vi "Create Error (ID).vi"(4 "timestamp? (True)":bool=TRUE, 5 "is warning? (False)":bool, 6 "error override? (False)":bool, 7 "arg. call chain? (True)":bool=TRUE, 8 "error in (no error)":errorcluster, 9 "error arguments (\"\")":string, 10 "error description (\"\")":string, 11 "error id":string) -> (0 "error out":errorcluster)   [LabVIEW 2019, in "Error Generation.lvlib"]
doc: "Creates an error with an error ID instead of an error code. (Internally code = 637237 is used)\nThis function is similar to original NI \"Error Cluster From Error Code.vi\". Additional functions:\n<b>timestamp?</b>\nadd a current date & time string to the error description.\n<b>error override?</b>\nOverride the error on the input with the error code, despriction & arguments. \n<b>error arguments</b>\nInsert an argument name and data in this format: argument=argument data\nMultiple Arguments can be inserted EOL separated.\nUse arguments, to specify the error more detailled.\n- - -\nCopyright (c) 2023, Merecs Engineering GmbH"
uses:
  Error Generation.lvlib
  <vilib>/Utility/error.llb/Clear Errors.vi
  support/Convert Argument Representation.vi
  support/Search and Replace String With Arguments.vi
  Add Error Description.vi
  Get Argument.vi
  support/Is Error Code.vi
  support/Error Cluster From Error Code (Merecs).vi
  String to Match Pattern Case Insensitive.vi
  <vilib>/Utility/error.llb/Trim Whitespace.vi
  <vilib>/Utility/error.llb/Check Special Tags.vi
panel:
  # "Connector Pane"
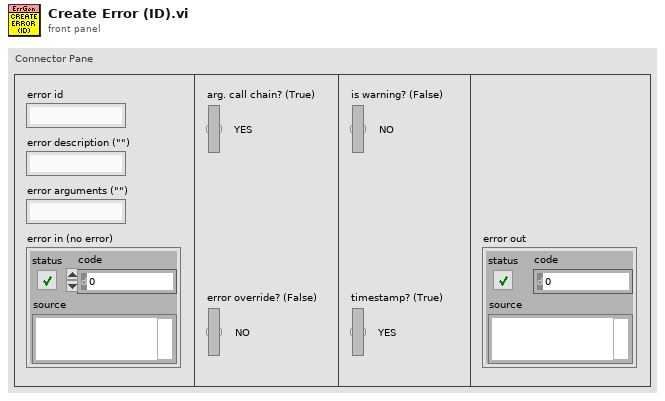
[diagram p1: front panel]
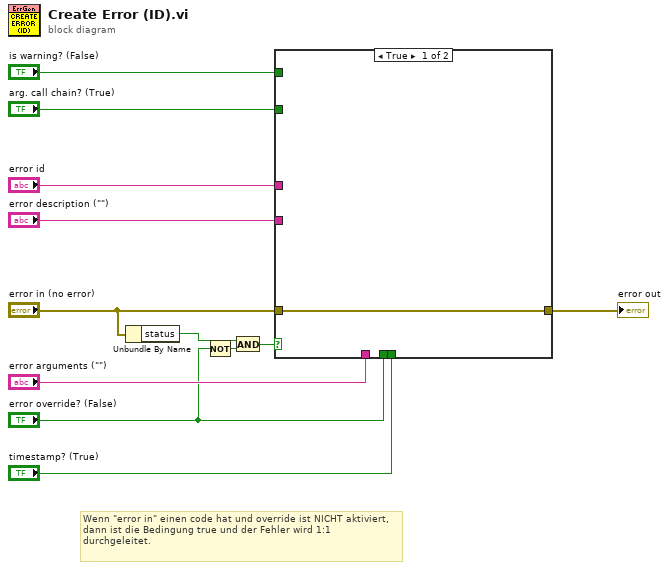
[diagram p0: block diagram]
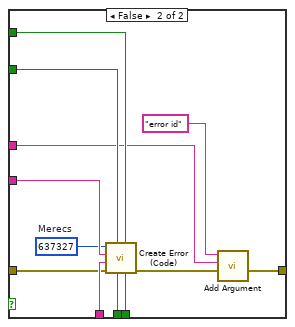
[diagram p2: hidden frame]
diagram:
  # "Wenn \"error in\" einen code hat und override ist NICHT aktiviert, dann ist die Bedingung true und der Fehler wird 1:1 durchgeleitet."
  n1 = Unbundle By Name("error in (no error)") -> ("status"=w4:bool)
  n2 = Not(x="error override? (False)") -> (.not. x?=w2:bool)
  n3 = And(x=w4, y=w2) -> (x .and. y?=w1:bool)
  n4 = case shown="True" w1 {
    tunnel: "error arguments (\"\")" -> [_ w24]
    tunnel: "error description (\"\")" -> [_ w23]
    tunnel: "error override? (False)" -> [_ w22]
    tunnel: "timestamp? (True)" -> [_ w21]
    tunnel: "arg. call chain? (True)" -> [_ w19]
    tunnel: "is warning? (False)" -> [_ w18]
    tunnel: "error in (no error)" -> [w13 w17]
    tunnel: [w13 w16] -> w7
    tunnel: "error id" -> [_ w15]
    frame True {
    }
    frame False {
      w20 = 637327  # Merecs
      n5 = call "Create Error (Code).vi"("timestamp? (True)"=w21, "is warning? (False)"=w18, "error override? (True)"=w22, "arg. call chain? (False)"=w19, "error in (no error)"=w17, "error arguments (\"\")"=w24, "error description (\"\")"=w23, "error code"=w20) -> ("error out"=w25:errorcluster)  [unwired: 3 in]
      n6 = call "Add Argument.vi"("error in (no error)"=w25, "argument data"=w15, "argument"="error id") -> ("error out"=w16:errorcluster)  [unwired: 8 in]
    }
  }
  "error out" <- w7
